vi "Own20261013_ScriptingAdd_V2.vi"() -> ()   [LabVIEW 2024]
uses:
  development/opensource-native_f4d362723206446591f3edf72d9fd4e8/source/library/Scripting.lvlib
panel:
  out "error out":errorcluster
  out "terminal_id":u32
  in  "source_y":u32
  in  "source_x":u32
  in  "owner_diagram_id":u32
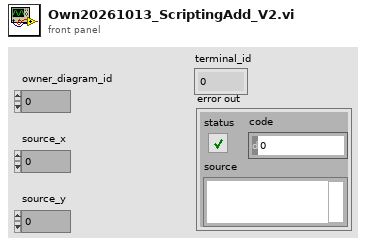
[diagram p1: front panel]
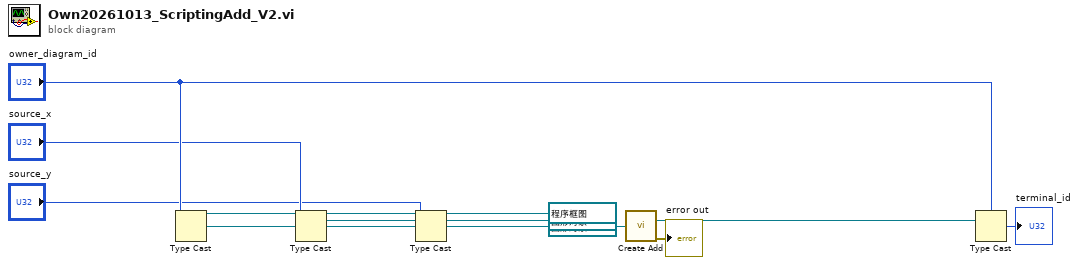
[diagram p0: block diagram]
diagram:
  n1 = Type Cast(type=refnum<vi> refnum ("Diagram in"), x="owner_diagram_id") -> (*(type *) &x=w10:refnum<vi>)
  n2 = Type Cast(type=refnum<vi> refnum ("x"), x="source_x") -> (*(type *) &x=w7:refnum<vi>)
  n3 = Type Cast(type=refnum<vi> refnum ("y"), x="source_y") -> (*(type *) &x=w4:refnum<vi>)
  n4 = call "Create Add.vi"("Diagram in"=w10, "x"=w7, "y"=w4) -> ("x+y"=w3:refnum<vi>, "error out"=→"error out":errorcluster)  [unwired: 10 in, 1 out]
  n5 = Type Cast(type="owner_diagram_id", x=w3) -> (*(type *) &x=→"terminal_id":u32)
